vi "Write to Text File (with Core and Type).vi"(0 "Database Filepath (xlsx)":path=path "C:/Users/jkreienh/Desktop/Preliminary Ballard Database Template.xlsx", 2 "Filetype":enum16{"Hardware", "Parameter"}(ring), 5 "Core":i32, 7 "Text":string, 11 "Error (in)":errorcluster) -> (15 "Error (out)":errorcluster)   [LabVIEW 2020]
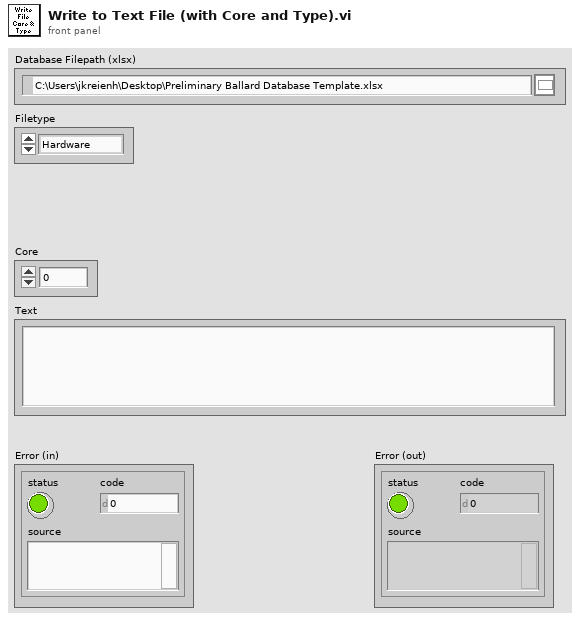
[diagram p1: front panel]
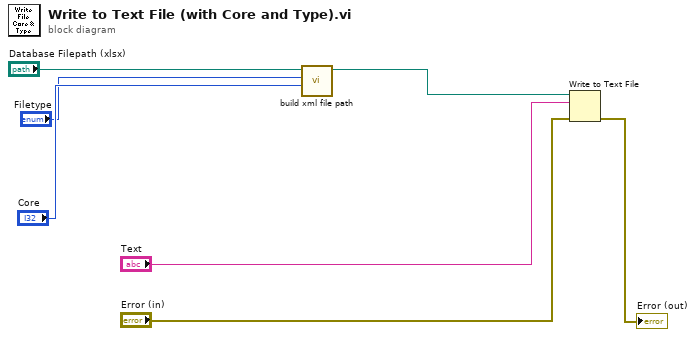
[diagram p0: block diagram]
diagram:
  n1 = call "build xml file path.vi"("Core"="Core", "Filetype"="Filetype", "Database Filepath in"="Database Filepath (xlsx)") -> ("xml path out"=w4:path)  [unwired: 8 in]
  n2 = Write to Text File(file (use dialog)=w4, text="Text", error in="Error (in)") -> (error out=→"Error (out)":errorcluster)  [unwired: 1 in, 2 out]
